vi "Nom regulateur.vi"(2 "Adresse régulateur":u8, 3 "Port COM run 1 REG":refnum<visa-resource-name> caption="Port RS232") -> (1 "Nom régulateur":string)   [LabVIEW 2022 SP3]
uses:
  Variables globales/Variables glob EUROTHERM.vi
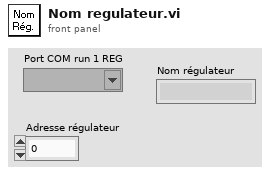
[diagram p1: front panel]
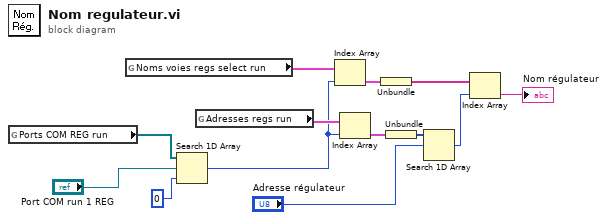
[diagram p0: block diagram]
diagram:
  n1 = global read "Variables glob EUROTHERM.vi" "Ports COM REG run"() -> (w4:refnum<visa-resource-name>[])
  n2 = global read "Variables glob EUROTHERM.vi" "Noms voies regs select run"() -> (w5:cluster{"Noms voies select run 1COM":string[]}[])
  n3 = Search 1D Array(1D array=w4, element="Port COM run 1 REG", start index (0)=0 ("indice de départ (0)")) -> (index of element=w1:i32)
  n4 = global read "Variables glob EUROTHERM.vi" "Adresses regs run"() -> (w7:cluster{"Adresses run 1COM reg":u16[]}[])
  n5 = Index Array(array=w5, index=w1) -> (element=w6:cluster{"Noms voies select run 1COM":string[]})
  n6 = Index Array(array=w7, index=w1) -> (element=w8:cluster{"Adresses run 1COM reg":u16[]})
  n7 = Unbundle(w6) -> ("Noms voies select run 1COM"=w11:string[])
  n8 = Unbundle(w8) -> ("Adresses run 1COM reg"=w9:u16[])
  n9 = Search 1D Array(1D array=w9, element="Adresse régulateur") -> (index of element=w12:i32)  [unwired: 1 in]
  n10 = Index Array(array=w11, index=w12) -> (element=→"Nom régulateur":string)
